vi "ZM-HW-do.vi"(8 "error in (no error)":errorcluster, 11 "ZM-HW-hardware in":refnum<class "ZM-HW-hardware.lvclass">) -> (0 "error out":errorcluster, 2 "package":refnum<class "ZM-PC-package.lvclass">, 3 "ZM-HW-hardware out":refnum<class "ZM-HW-hardware.lvclass">)   [LabVIEW 2020, in "ZM-HW-hardware.lvlib" / "ZM-HW-hardware.lvclass"]
doc: "Placeholder: returns a default package and error 5000 (#customerror 5000). A child class must override it. The package out is a default ZM-PC-package object; the error is built by Bundle By Name onto an error-cluster constant (status TRUE, code 5000, source ZM-HW-do.vi: must be overridden by a child class) and merged after error in, so an incoming error wins."
uses:
  ZM-HW-hardware.lvclass
  common/ZM-PC-packages/ZM-PC-package/ZM-PC-package.lvclass
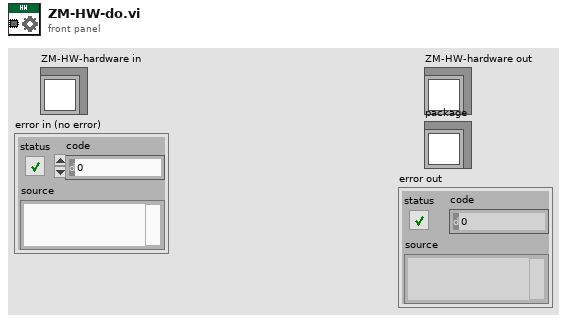
[diagram p1: front panel]
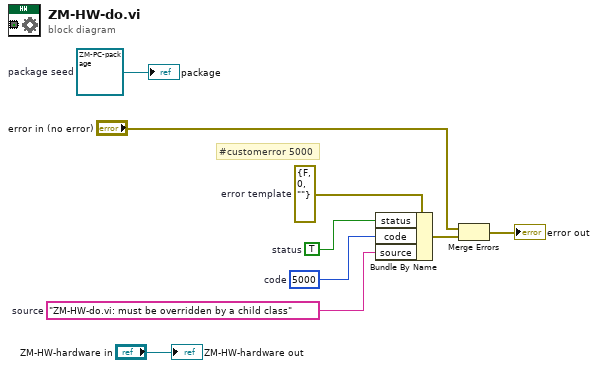
[diagram p0: block diagram]
diagram:
  w7 = "ZM-HW-do.vi: must be overridden by a child class"  # source
  w8 = 5000  # code
  w9 = TRUE  # status
  w6 = errorcluster {"status"=FALSE, "code"=0, "source"=""}  # error template
  w2 = refnum<class "ZM-PC-package.lvclass"> refnum  # package seed
  # "#customerror 5000"
  n1 = Bundle By Name(cluster=w6, "status"=w9, "code"=w8, "source"=w7) -> (w4:errorcluster)
  n2 = Merge Errors("error in (no error)", w4) -> (→"error out":errorcluster)
  "ZM-HW-hardware out" <- "ZM-HW-hardware in"
  "package" <- w2
